vi "Eval_MultiVar_MultiRes.vi"(8 "error in (no error)":errorcluster, 9 "varValues":dbl[](array[numeric]) format="%#_13g", 10 "varNames":string[](array[string]), 11 "muExpr in":refnum<class "mupExpr.lvclass">) -> (0 "error out":errorcluster, 2 "Results":dbl[](array[numeric]) format="%#_13g", 3 "muExpr out":refnum<class "mupExpr.lvclass">)   [LabVIEW 2015, in "mupExpr.lvclass"]
doc: "Update the value of multiple variables then evaluate the expression.\nReturns one result per expression.\n\nIf the expressions contain no variables, the input values are ignored.\n\nIf the variables are defined for bulk mode evaluation, only the first set (index 0) will be updated and evaluated."
uses:
  mupExpr.lvclass
  mupExpr.lvclass/mupExpr.ctl
  mupLib/mupSetVarValue.vi
  mupLib/mupCheckError.vi
  <vilib>/Utility/error.llb/Error Cluster From Error Code.vi
  mupLib/mupLib.lvlib
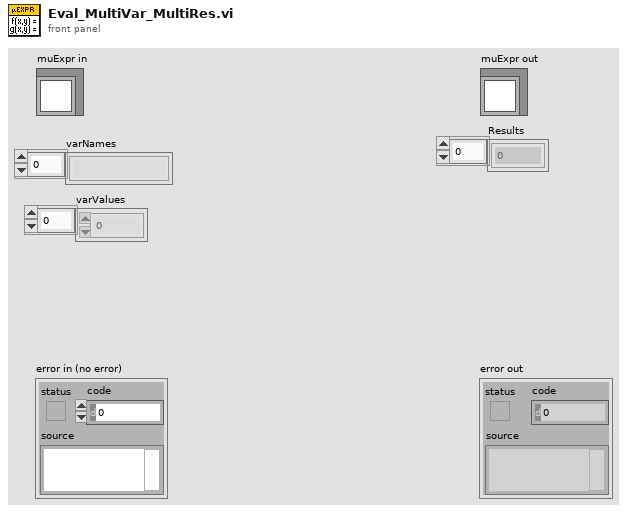
[diagram p1: front panel]
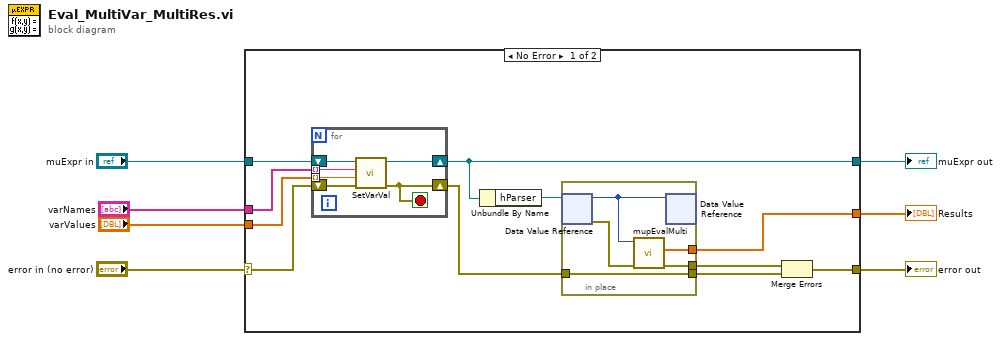
[diagram p0: block diagram]
diagram:
  n1 = case shown="No Error" "error in (no error)" {
    selector: "error in (no error)" -> [w14 w31]
    tunnel: "varValues" -> [w15 _]
    tunnel: "varNames" -> [w16 _]
    tunnel: [w9 _] -> w5
    tunnel: "muExpr in" -> [w17 w30]
    tunnel: [w18 w31] -> w3
    tunnel: [w8 w30] -> w2
    frame No Error {
      n2 = for {
        tunnel: w16 -> [w29] mode=indexing
        tunnel: w15 -> [w28] mode=indexing
        shift-right: [w24] -> w12
        shift-left: w14 -> [w27]
        shift-right: [w25] -> w8
        shift-left: w17 -> [w26]
        stop <- w24 stop-if-true
        n3 = call "SetVarVal.vi"("error in (no error)"=w27, "varValue"=w28, "varName"=w29, "muExpr in"=w26) -> ("error out"=w24:errorcluster, "muExpr out"=w25:refnum<class "mupExpr.lvclass">)  [unwired: 6 in]
      }
      n4 = Unbundle By Name(w8) -> ("hParser"=w13:refnum<data-value>)
      n5 = in-place {
        in-place-border: w12 -> [w22]
        in-place-border: [w23] -> w11
        in-place-border: [w21] -> w9
        in-place-border: [w22] -> w10
        n6 = in-place-dvr #1(w13) -> (w19:u64, w20:errorcluster)
        n7 = call "mupEvalMulti.vi"("error in (no error)"=w20, "hParser in"=w19) -> ("error out"=w23:errorcluster, "results"=w21:dbl[])  [unwired: 6 in, 2 out]
        n8 = in-place-dvr #1(w19) -> ()  [unwired: 2 out]
      }
      n9 = Merge Errors(w11, w10) -> (w18:errorcluster)
    }
    frame Error {
    }
  }
  "error out" <- w3
  "muExpr out" <- w2
  "Results" <- w5
